vi "GOOP_VirtualFolder_Item_OnCommand.vi"(10 "Command Tag":string, 11 "Object":u64) -> ()   [LabVIEW 2020]
uses:
  <resource>/Framework/Providers/Open_GDS/ClassProviders/Provider_BaseClassInterface/ClassWriter_class/ClassWriter.lvclass
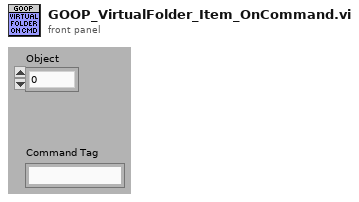
[diagram p1: front panel]
types:
  T1 = enum8{"No dynamic dispatch VIs", "Include nearest implementation", "Include all overrides"}
  T2 = typedef "GDSIconEditor_FileNameFilter.ctl" = cluster{"String/Match Pattern to remove":string[], "Strings To Convert From - To":cluster{"From":string, "To":string}[]}
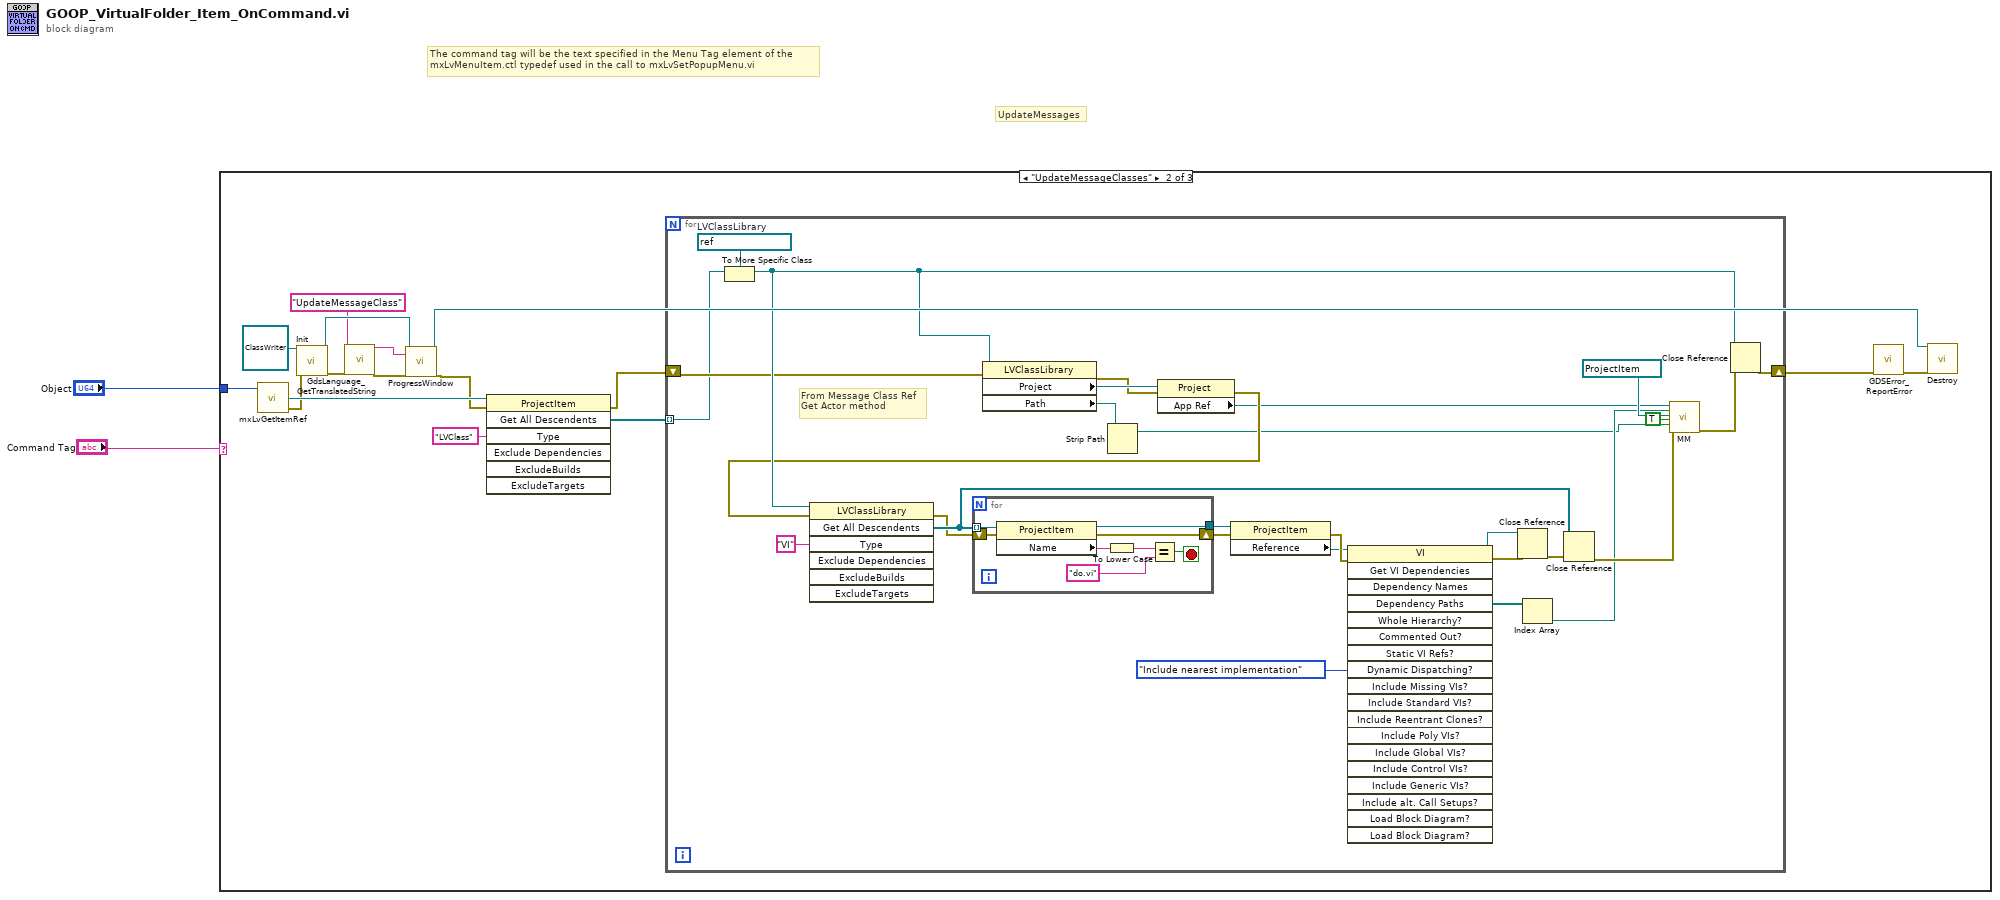
[diagram p0: block diagram]
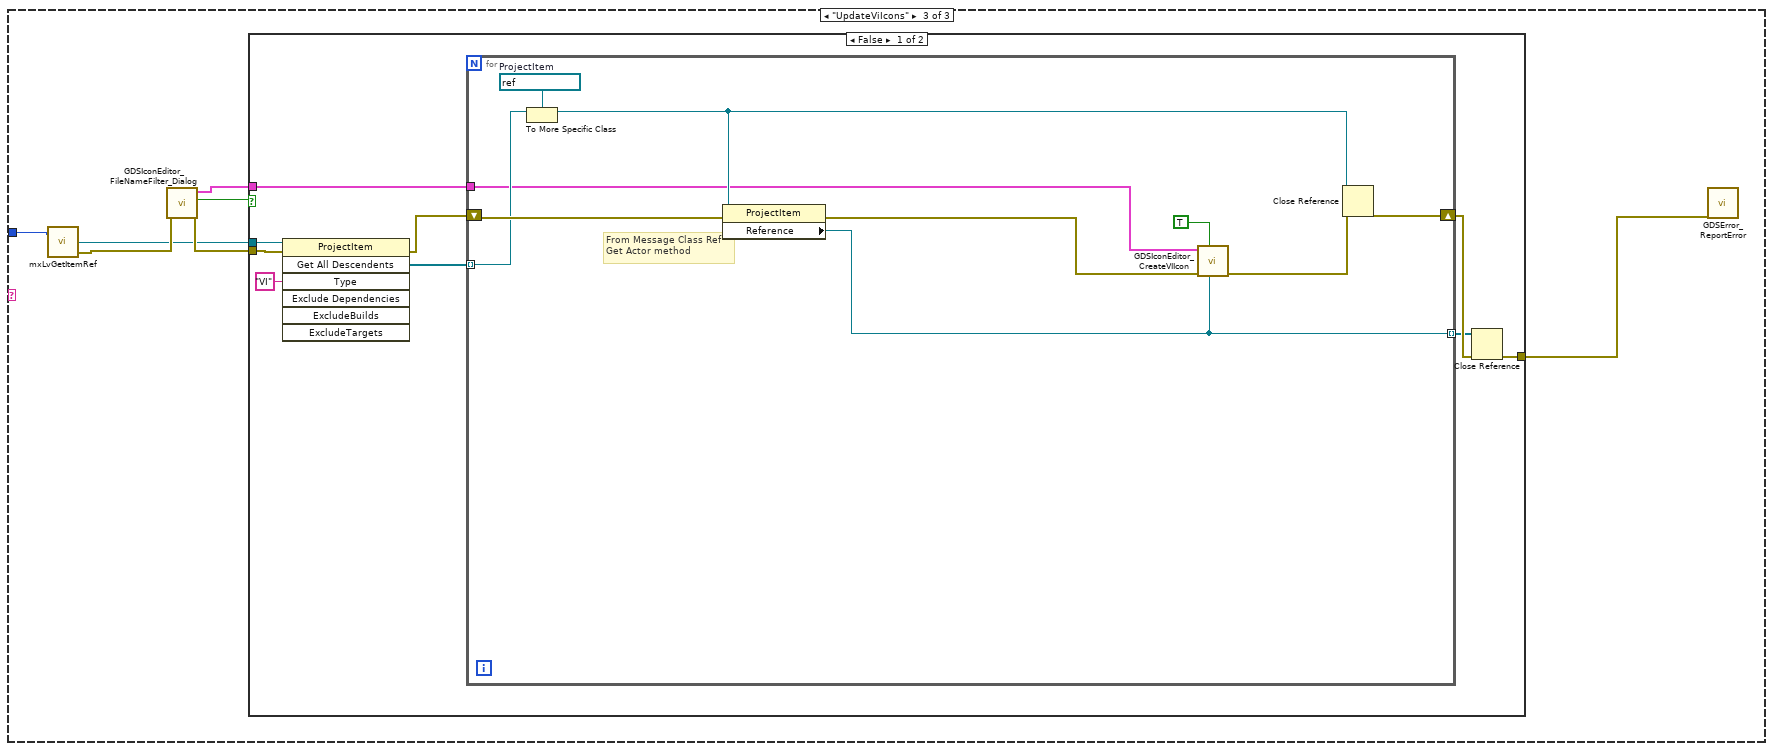
[diagram p3: hidden frame]
diagram:
  # "UpdateMessages"
  # "The command tag will be the text specified in the Menu Tag element of the \nmxLvMenuItem.ctl typedef used in the call to mxLvSetPopupMenu.vi"
  n1 = case shown="\"UpdateMessageClasses\"" "Command Tag" {
    tunnel: "Object" -> [_ w18 w61]
    frame Default {
    }
    frame "UpdateMessageClasses" {
      n2 = call <resource>:"mxLvGetItemRef.vi"("Item"=w18) -> ("Item Refnum"=w17:refnum<vi>, "error out"=w6:errorcluster)  [unwired: 1 in, 1 out]
      n3 = call-dynamic "Init.vi"("ClassWriter in"=refnum<class "ClassWriter.lvclass"> refnum, "error in (no error)"=w6) -> ("ClassWriter out"=w14:refnum<class "ClassWriter.lvclass">, "error out"=w11:errorcluster)  [unwired: 16 in]
      n4 = call <resource>:"GdsLanguage_GetTranslatedString.vi"("StringID(s)"="UpdateMessageClass" ("Message(Exit)"), "error in (no error)"=w11) -> ("FirstStringOut"=w10:string, "error out"=w12:errorcluster)  [unwired: 14 in, 2 out]
      n5 = call-dynamic "ProgressWindow.vi"("ClassWriter in"=w14, "Message(Exit)"=w10, "error in (no error)"=w12) -> ("ClassWriter out"=w15:refnum<class "ClassWriter.lvclass">, "error out"=w4:errorcluster)  [unwired: 15 in]
      n6 = invoke class="ProjectItem" method="Get All Descendents"(reference=w17, error in=w4, "Type"="LVClass") -> (error out=w5:errorcluster, "All Descendents"=w7:refnum<vi>[])  [unwired: 4 in, 5 out]
      n7 = for {
        tunnel: w7 -> [w19] mode=indexing
        shift-right: [w21] -> w8
        shift-left: w5 -> [w44]
        w20 = refnum<vi> refnum  # LVClassLibrary
        # "From Message Class Ref\nGet Actor method"
        n8 = To More Specific Class(target class=w20, reference=w19) -> (specific class reference=w45:refnum<vi>)  [unwired: 1 in, 1 out]
        n9 = property class="LVClassLibrary"(reference=w45, error in=w44) -> (error out=w22:errorcluster, "Project"=w23:refnum<vi>, "Path"=w26:path)  [unwired: 1 out]
        n10 = Strip Path(path=w26) -> (stripped path=w27:path)  [unwired: 1 out]
        n11 = property class="Project"(reference=w23, error in=w22) -> (error out=w33:errorcluster, "App Ref"=w24:refnum<vi>)  [unwired: 1 out]
        n12 = invoke class="LVClassLibrary" method="Get All Descendents"(reference=w45, error in=w33, "Type"="VI") -> (error out=w31:errorcluster, "All Descendents"=w39:refnum<vi>[])  [unwired: 4 in, 5 out]
        n13 = for {
          tunnel: w39 -> [w54] mode=indexing
          tunnel: [w50] -> w29
          shift-right: [w49] -> w30
          shift-left: w31 -> [w48]
          stop <- w47 stop-if-true
          n14 = property class="ProjectItem"(reference=w54, error in=w48) -> (reference out=w50:refnum<vi>, error out=w49:errorcluster, "Name"=w53:string)
          n15 = To Lower Case(string=w53) -> (all lower case string=w52:string)
          n16 = Equal?(x=w52, y="do.vi") -> (x = y?=w47:bool)
        }
        n17 = property class="ProjectItem"(reference=w29, error in=w30) -> (error out=w35:errorcluster, "Reference"=w32:refnum<vi>)  [unwired: 1 out]
        n18 = invoke class="VI" method="Get VI Dependencies"(reference=w32, error in=w35, "Dynamic Dispatching?"=T1."Include nearest implementation") -> (reference out=w37:refnum<vi>, error out=w36:errorcluster, "Dependency Paths"=w40:path[])  [unwired: 16 in, 16 out]
        n19 = Close Reference(reference=w37, error in (no error)=w36) -> (error out=w38:errorcluster)
        n20 = Index Array(array=w40) -> (element=w41:path)  [unwired: 1 in]
        n21 = Close Reference(reference=w39, error in (no error)=w38) -> (error out=w42:errorcluster)
        n22 = call <resource>:"MM.vi"("AppInst"=w24, "ActorMethod"=w41, "ActorClassItemRef(Don't Delete)"=refnum<vi> refnum, "OnlyUpdate(if needed,False)"=TRUE ("OnlyUpdate(if needed)"), "Destination Path"=w27, "error in"=w42) -> ("error out"=w43:errorcluster)  [unwired: 13 in]
        n23 = Close Reference(reference=w45, error in (no error)=w43) -> (error out=w21:errorcluster)
      }
      n24 = call <resource>:"GDSError_ReportError.vi"("error in (no error)"=w8) -> ("error out"=w13:errorcluster)  [unwired: 18 in]
      n25 = call-dynamic "Destroy.vi"("ClassWriter.lvclass"=w15, "error in (no error)"=w13) -> ()  [unwired: 17 in, 1 out]
    }
    frame "UpdateViIcons" {
      n26 = call <resource>:"mxLvGetItemRef.vi"("Item"=w61) -> ("Item Refnum"=w58:refnum<vi>, "error out"=w60:errorcluster)  [unwired: 1 in, 1 out]
      n27 = call <resource>:"GDSIconEditor_FileNameFilter_Dialog.vi"("error in"=w60) -> ("error out"=w59:errorcluster, "Cancelled"=w57:bool, "FileNameConverions"=w55:T2)  [unwired: 8 in]
      n28 = case shown="False" w57 {
        tunnel: w59 -> [w67 w81]
        tunnel: w58 -> [w66 _]
        tunnel: [w63 w81] -> w56
        tunnel: w55 -> [w62 _]
        frame False {
          n29 = invoke class="ProjectItem" method="Get All Descendents"(reference=w66, error in=w67, "Type"="VI") -> (error out=w68:errorcluster, "All Descendents"=w69:refnum<vi>[])  [unwired: 4 in, 5 out]
          n30 = for {
            tunnel: w69 -> [w76] mode=indexing
            shift-right: [w78] -> w65
            shift-left: w68 -> [w79]
            tunnel: [w73] -> w64 mode=indexing
            tunnel: w62 -> [w71]
            w77 = refnum<vi> refnum  # ProjectItem
            # "From Message Class Ref\nGet Actor method"
            n31 = To More Specific Class(target class=w77, reference=w76) -> (specific class reference=w80:refnum<vi>)  [unwired: 1 in, 1 out]
            n32 = property class="ProjectItem"(reference=w80, error in=w79) -> (error out=w72:errorcluster, "Reference"=w73:refnum<vi>)  [unwired: 1 out]
            n33 = call <resource>:"GDSIconEditor_CreateVIIcon.vi"("ViRef(IgnoreIfNotWired)"=w73, "AutomaticUpdateNoQuestionsAsked(False)"=TRUE, "error in (no error)"=w72, "FileNameConverions"=w71) -> ("error out"=w74:errorcluster)  [unwired: 7 in]
            n34 = Close Reference(reference=w80, error in (no error)=w74) -> (error out=w78:errorcluster)
          }
          n35 = Close Reference(reference=w64, error in (no error)=w65) -> (error out=w63:errorcluster)
        }
        frame True {
        }
      }
      n36 = call <resource>:"GDSError_ReportError.vi"("error in (no error)"=w56) -> ()  [unwired: 18 in, 1 out]
    }
  }
